vi "Main.vi"() -> ()   [LabVIEW 2026]
doc: "This template is for the Queued Message Handler design pattern.\n\nThe Event Handling Loop generates messages based on user interface actions.\n\nThe Message Handling Loop processes messages generated by the Event Handling Loop, or by other messages. The messages are string values, so new messages can be added easily to the Message Cases case structure in the Message Handling Loop. Each message cluster can also provide an optional value for Message Data, which is a variant that can be converted to whatever message-specific data is required."
uses:
  controls/UI Data.ctl
  support/Message Queue/Enqueue Message (Single).vi
  <vilib>/Utility/error.llb/Error Cluster From Error Code.vi
  <vilib>/ErrorRing/Error Ring.xnode
  support/Message Queue/Message Queue.lvlib
  support/User Event - Stop/User Event - Stop.lvlib
panel:
  out "Slide":dbl(slide) scale=0.0..100.0
  out "Meter":dbl(knob) scale=0.0..10.0
  in  "Volts":dbl(knob) scale=0.0..10.0
  out "Display <Replace Me>":string
  in  "Do Something Else <Replace Me>":bool
  in  "Do Something <Replace Me>":bool
  in  "Exit":bool
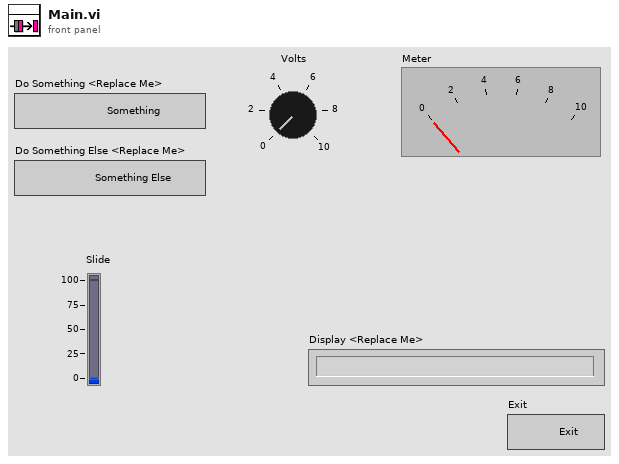
[diagram p1: front panel]
types:
  T1 = typedef "UI Data.ctl" = cluster{"Boolean <Replace Me>":bool, "String <Replace Me>":string, "Numeric <Replace Me>":dbl, "Do Something Ref":refnum<vi>, "Do Something Else Ref":refnum<vi>, "Data Display Ref":refnum<vi>, "Exit Button Ref":refnum<vi>}
  T2 = typedef "Message Queue.lvlib/All Message Queues.ctl" = cluster{"UI":refnum<queue>}
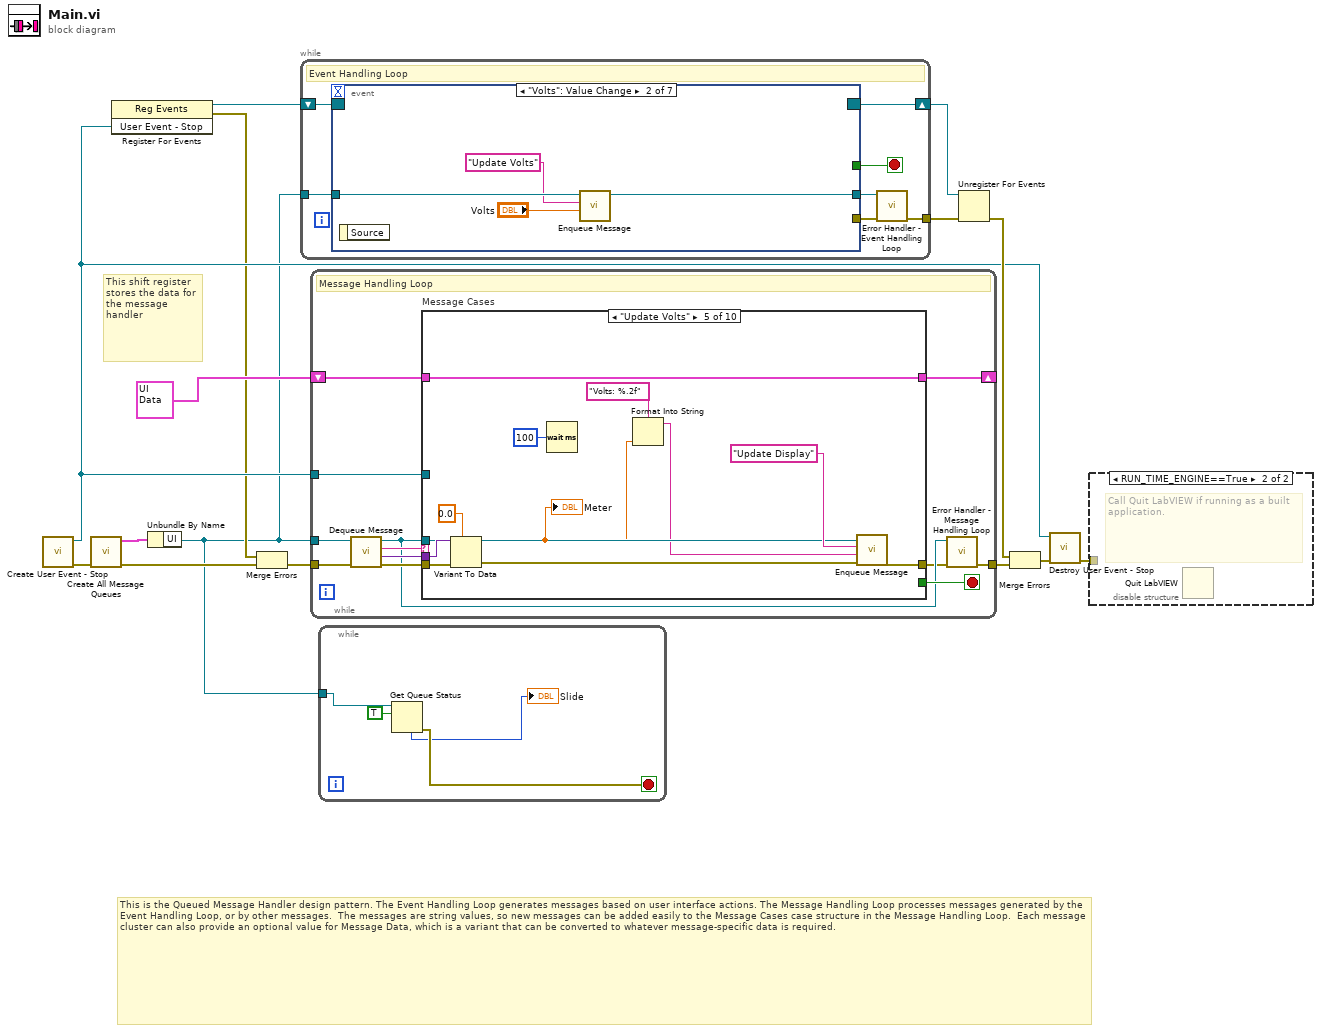
[diagram p0: block diagram]
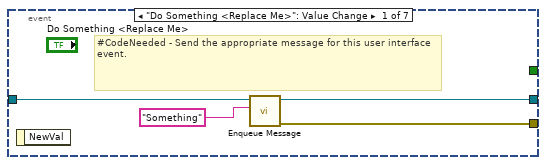
[diagram p3: hidden frame]
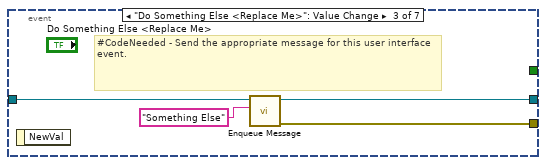
[diagram p4: hidden frame]
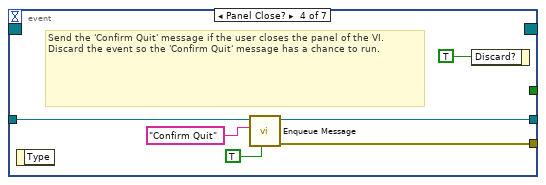
[diagram p5: hidden frame]
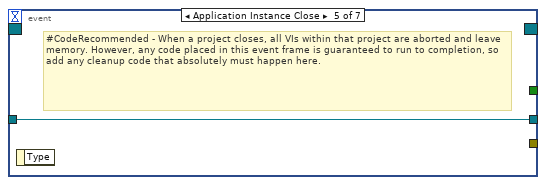
[diagram p6: hidden frame]
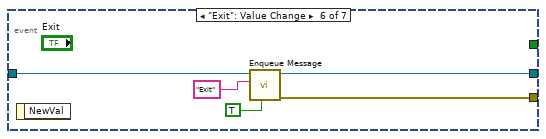
[diagram p7: hidden frame]
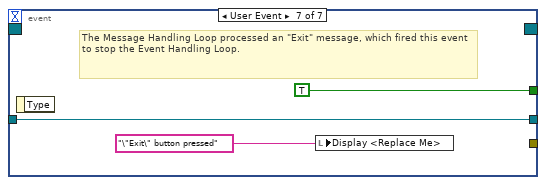
[diagram p8: hidden frame]
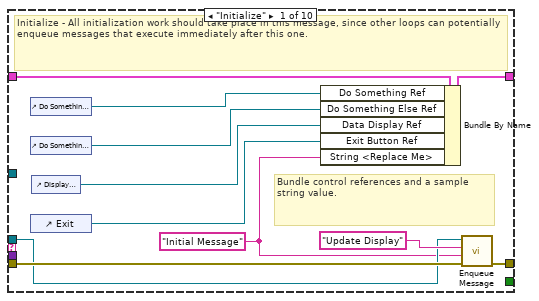
[diagram p9: hidden frame]
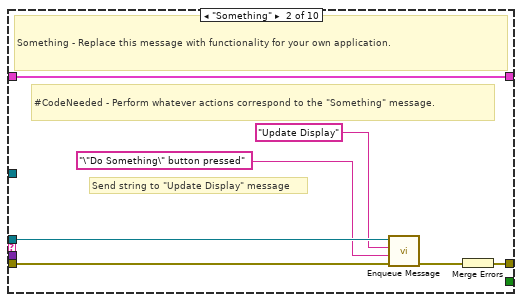
[diagram p10: hidden frame]
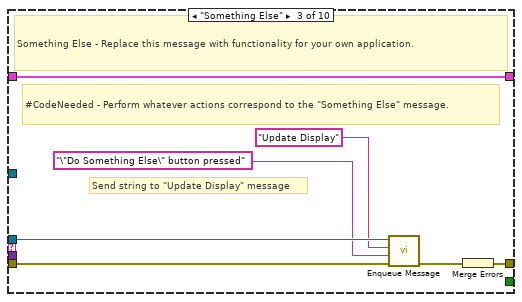
[diagram p11: hidden frame]
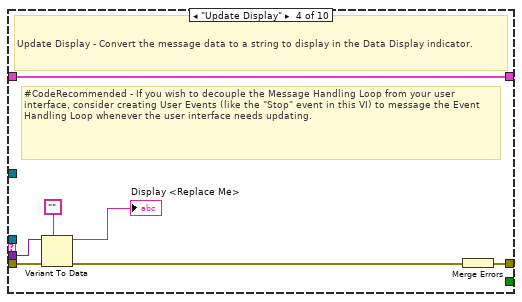
[diagram p12: hidden frame]
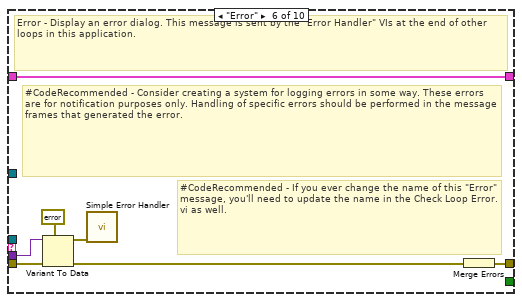
[diagram p13: hidden frame]
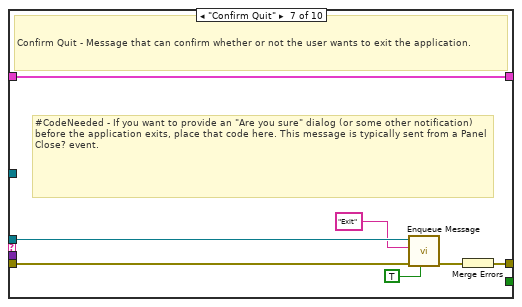
[diagram p14: hidden frame]
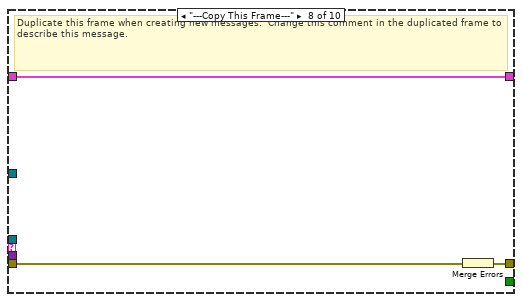
[diagram p15: hidden frame]
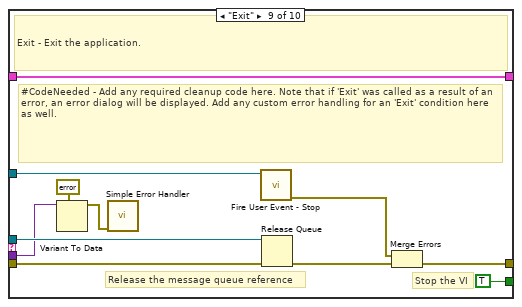
[diagram p16: hidden frame]
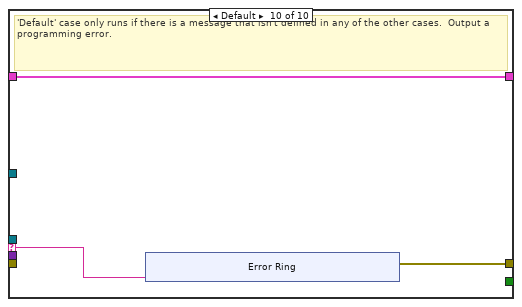
[diagram p17: hidden frame]
diagram:
  # "This is the Queued Message Handler design pattern. The Event Handling Loop generates messages based on user interface actions. The Message Handling Loop processes messages generated by the Event Handling Loop, or by other messages.  The messages are string values, so new messages can be added easily to the Message Cases case structure in the Message Handling Loop.  Each message cluster can also provide an optional value for Message Data, which is a variant that can be converted to whatever message-specific data is required."
  # "This shift register stores the data for the message handler"
  n1 = call "Create User Event - Stop.vi"() -> ("error out"=w12:errorcluster, "User Event - Stop"=w4:refnum<user-event>)  [unwired: 10 in]
  n2 = call "Create All Message Queues.vi"("error in (no error)"=w12) -> ("error out"=w15:errorcluster, "Message Queues out"=w14:T2)  [unwired: 9 in]
  n3 = register-events(w4) -> (reference out=w5:refnum<event-registration>, error out=w2:errorcluster)  [unwired: 2 in]
  n4 = Unbundle By Name(w14) -> ("UI"=w1:refnum<queue>)
  n5 = Merge Errors(w2, w15) -> (w3:errorcluster)
  n6 = while {
    tunnel: w1 -> [w22]
    shift-right: [w20] -> w9
    shift-left: w5 -> [w21]
    tunnel: [w16] -> w6
    stop <- w18 stop-if-true
    # "Event Handling Loop"
    n7 = event shown="[1] \"Volts\": Value Change" {
      selector: w21 -> [_ _ _ _ _ _ _]
      dyn-events: [_ _ _ _ _ _ _] -> w20
      timeout: _ -> [_ _ _ _ _ _ _]
      tunnel: [_ _ _ _ _ _ TRUE ("Discard?")] -> w18
      tunnel: w22 -> [w26 w30 w34 w39 w41 w46 w49]
      tunnel: [w23 _ w31 w38 _ w45 _] -> w19
      tunnel: [w25 w29 w33 w37 w41 w44 w49] -> w17
      event "Do Something <Replace Me>": Value Change {
        # "#CodeNeeded - Send the appropriate message for this user interface event."
        n8 = event-data() -> ()  [unwired: 1 in, 1 out]
        n9 = call-poly "Enqueue Message.vi"("Message"="Something", "Message Queue"=w26) -> ("error out"=w23:errorcluster, "dup Message Queue"=w25:refnum<queue>)  [unwired: 8 in]
      }
      event "Volts": Value Change {
        n10 = event-data() -> ()  [unwired: 1 in, 1 out]
        n11 = call-poly "Enqueue Message.vi"("Message Data"="Volts", "Message"="Update Volts", "Message Queue"=w30) -> ("dup Message Queue"=w29:refnum<queue>)  [unwired: 7 in, 1 out]
      }
      event "Do Something Else <Replace Me>": Value Change {
        # "#CodeNeeded - Send the appropriate message for this user interface event."
        n12 = event-data() -> ()  [unwired: 1 in, 1 out]
        n13 = call-poly "Enqueue Message.vi"("Message"="Something Else", "Message Queue"=w34) -> ("error out"=w31:errorcluster, "dup Message Queue"=w33:refnum<queue>)  [unwired: 8 in]
      }
      event Panel Close? {
        # "Send the 'Confirm Quit' message if the user closes the panel of the VI. Discard the event so the 'Confirm Quit' message has a chance to run."
        n14 = event-data() -> ()  [unwired: 1 in, 1 out]
        n15 = call-poly "Enqueue Message.vi"("Priority Message? (F)"=TRUE, "Message"="Confirm Quit", "Message Queue"=w39) -> ("error out"=w38:errorcluster, "dup Message Queue"=w37:refnum<queue>)  [unwired: 7 in]
        n16 = event-data("Discard?"=TRUE) -> ()  [unwired: 1 in, 1 out]
      }
      event Application Instance Close {
        # "#CodeRecommended - When a project closes, all VIs within that project are aborted and leave memory. However, any code placed in this event frame is guaranteed to run to completion, so add any cleanup code that absolutely must happen here."
        n17 = event-data() -> ()  [unwired: 1 in, 1 out]
      }
      event "Exit": Value Change {
        n18 = event-data() -> ()  [unwired: 1 in, 1 out]
        n19 = call-poly "Enqueue Message.vi"("Priority Message? (F)"=TRUE, "Message"="Exit", "Message Queue"=w46) -> ("error out"=w45:errorcluster, "dup Message Queue"=w44:refnum<queue>)  [unwired: 7 in]
      }
      event User Event {
        # "The Message Handling Loop processed an \"Exit\" message, which fired this event to stop the Event Handling Loop."
        n20 = event-data() -> ()  [unwired: 1 in, 1 out]
        n21 = local write "Display <Replace Me>"("\"Exit\" button pressed" ("VI Stopped")) -> ()
      }
    }
    n22 = call "Error Handler - Event Handling Loop.vi"("error in (no error)"=w19, "Message Queue"=w17) -> ("dup error in"=w16:errorcluster)  [unwired: 8 in, 1 out]
  }
  n23 = while {
    tunnel: w1 -> [w53]
    shift-right: [w60] -> _
    shift-left: T1 {"Boolean <Replace Me>"=FALSE, "String <Replace Me>"="", "Numeric <Replace Me>"=0.0, "Do Something Ref"=refnum, "Do Something Else Ref"=refnum, "Data Display Ref"=refnum, "Exit Button Ref"=refnum} ("Data Cluster") -> [w61]
    tunnel: w4 -> [w58]
    tunnel: w3 -> [w57]
    tunnel: [w51] -> w13
    stop <- w59 stop-if-true
    # "Message Handling Loop"
    n24 = call "Dequeue Message.vi"("error in (no error)"=w57, "Message Queue"=w53) -> ("error out"=w56:errorcluster, "Message Data"=w54:variant, "Message"=w55:string, "dup Message Queue"=w52:refnum<queue>)  [unwired: 6 in]
    n25 = case "Message Cases" shown="\"Update Volts\"" w55 {
      selector: w55 -> [_ _ _ _ _ _ _ _ _ w134]
      tunnel: w52 -> [w63 w75 w82 _ w98 _ w115 _ w133 _]
      tunnel: w56 -> [w71 w77 w84 w91 w105 w112 w119 w122 w126 _]
      tunnel: [w72 w78 w85 w92 w100 w106 w117 w120 w129 w135] -> w50
      tunnel: w61 -> [w70 w79 w86 w93 w104 w111 w118 w121 w132 w136]
      tunnel: [w69 w79 w86 w93 w104 w111 w118 w121 w132 w136] -> w60
      tunnel: [_ _ _ _ _ _ _ _ TRUE _] -> w59
      tunnel: w54 -> [_ _ _ w90 w103 w110 _ _ w123 _]
      tunnel: w58 -> [_ _ _ _ _ _ _ _ w128 _]
      frame "Initialize" {
        w62 = "Initial Message" ("Initial Message")
        # "Bundle control references and a sample string value."
        # "Initialize - All initialization work should take place in this message, since other loops can potentially enqueue messages that execute immediately after this one."
        n26 = control-ref of="Do Something <Replace Me>"() -> (w68:refnum<vi>)
        n27 = control-ref of="Do Something Else <Replace Me>"() -> (w67:refnum<vi>)
        n28 = control-ref of="Exit"() -> (w65:refnum<vi>)
        n29 = control-ref of="Display <Replace Me>"() -> (w66:refnum<vi>)
        n30 = Bundle By Name(cluster=w70, "Do Something Ref"=w68, "Do Something Else Ref"=w67, "Data Display Ref"=w66, "Exit Button Ref"=w65, "String <Replace Me>"=w62) -> (w69:T1)
        n31 = call-poly "Enqueue Message.vi"("error in (no error)"=w71, "Message Data"=w62, "Message"="Update Display", "Message Queue"=w63) -> ("error out"=w72:errorcluster)  [unwired: 6 in, 1 out]
      }
      frame "Something" {
        # "Send string to \"Update Display\" message"
        # "#CodeNeeded - Perform whatever actions correspond to the \"Something\" message."
        # "Something - Replace this message with functionality for your own application."
        n32 = call-poly "Enqueue Message.vi"("error in (no error)"=w77, "Message Data"="\"Do Something\" button pressed" ("\"Do Something\" button pressed"), "Message"="Update Display", "Message Queue"=w75) -> ("error out"=w76:errorcluster)  [unwired: 6 in, 1 out]
        n33 = Merge Errors(w76) -> (w78:errorcluster)
      }
      frame "Something Else" {
        # "Send string to \"Update Display\" message"
        # "#CodeNeeded - Perform whatever actions correspond to the \"Something Else\" message."
        # "Something Else - Replace this message with functionality for your own application."
        n34 = call-poly "Enqueue Message.vi"("error in (no error)"=w84, "Message Data"="\"Do Something Else\" button pressed" ("\"Do Something Else\" button pressed"), "Message"="Update Display", "Message Queue"=w82) -> ("error out"=w83:errorcluster)  [unwired: 6 in, 1 out]
        n35 = Merge Errors(w83) -> (w85:errorcluster)
      }
      frame "Update Display" {
        # "#CodeRecommended - If you wish to decouple the Message Handling Loop from your user interface, consider creating User Events (like the \"Stop\" event in this VI) to message the Event Handling Loop whenever the user interface needs updating."
        # "Update Display - Convert the message data to a string to display in the Data Display indicator."
        n36 = Variant To Data(error in=w91, type="", Variant=w90) -> (data=→"Display <Replace Me>":string, error out=w88:errorcluster)
        n37 = Merge Errors(w88) -> (w92:errorcluster)
      }
      frame "Update Volts" {
        n38 = Variant To Data(error in=w105, type=0.0, Variant=w103) -> (data=w96:dbl, error out=w99:errorcluster)
        "Meter" <- w96
        n39 = Wait (ms)(milliseconds to wait=u32 100) -> ()  [unwired: 1 out]
        n40 = Format Into String(format string="Volts: %.2f", w96) -> (resulting string=w97:string)  [unwired: 2 in, 1 out]
        n41 = call-poly "Enqueue Message.vi"("error in (no error)"=w99, "Message Data"=w97, "Message"="Update Display", "Message Queue"=w98) -> ("error out"=w100:errorcluster)  [unwired: 6 in, 1 out]
      }
      frame "Error" {
        # "#CodeRecommended - If you ever change the name of this \"Error\" message, you'll need to update the name in the Check Loop Error.vi as well."
        # "#CodeRecommended - Consider creating a system for logging errors in some way. These errors are for notification purposes only. Handling of specific errors should be performed in the message frames that generated the error."
        # "Error - Display an error dialog. This message is sent by the \"Error Handler\" VIs at the end of other loops in this application."
        n42 = Variant To Data(error in=w112, type=errorcluster {"status"=FALSE, "code"=0, "source"=""} ("error constant"), Variant=w110) -> (data=w108:errorcluster, error out=w107:errorcluster)
        n43 = call <vilib>:"Simple Error Handler.vi"("error in (no error)"=w108) -> ()  [unwired: 4 in, 5 out]
        n44 = Merge Errors(w107) -> (w106:errorcluster)
      }
      frame "Confirm Quit" {
        # "#CodeNeeded - If you want to provide an \"Are you sure\" dialog (or some other notification) before the application exits, place that code here. This message is typically sent from a Panel Close? event."
        # "Confirm Quit - Message that can confirm whether or not the user wants to exit the application."
        n45 = call-poly "Enqueue Message.vi"("Priority Message? (F)"=TRUE, "error in (no error)"=w119, "Message"="Exit", "Message Queue"=w115) -> ("error out"=w116:errorcluster)  [unwired: 6 in, 1 out]
        n46 = Merge Errors(w116) -> (w117:errorcluster)
      }
      frame "---Copy This Frame---" {
        # "Duplicate this frame when creating new messages.  Change this comment in the duplicated frame to describe this message."
        n47 = Merge Errors(w122) -> (w120:errorcluster)
      }
      frame "Exit" {
        # "Stop the VI"
        # "Release the message queue reference"
        # "#CodeNeeded - Add any required cleanup code here. Note that if 'Exit' was called as a result of an error, an error dialog will be displayed. Add any custom error handling for an 'Exit' condition here as well."
        # "Exit - Exit the application."
        n48 = Variant To Data(type=errorcluster {"status"=FALSE, "code"=0, "source"=""} ("error constant"), Variant=w123) -> (data=w124:errorcluster)  [unwired: 1 in, 1 out]
        n49 = call <vilib>:"Simple Error Handler.vi"("error in (no error)"=w124) -> ()  [unwired: 4 in, 5 out]
        n50 = call "Fire User Event - Stop.vi"("User Event - Stop"=w128) -> ("error out"=w127:errorcluster)  [unwired: 10 in]
        n51 = Release Queue(queue=w133, error in (no error)=w126) -> (error out=w130:errorcluster)  [unwired: 1 in, 2 out]
        n52 = Merge Errors(w127, w130) -> (w129:errorcluster)
      }
      frame Default {
        # "'Default' case only runs if there is a message that isn't defined in any of the other cases.  Output a programming error."
        n53 = xnode "Error Ring"("parameter 0"=w134) -> ("error out"=w135:errorcluster)
      }
    }
    n54 = call "Error Handler - Message Handling Loop.vi"("error in (no error)"=w50, "Message Queue"=w52) -> ("dup error in"=w51:errorcluster)  [unwired: 8 in, 1 out]
  }
  n55 = while {
    tunnel: w1 -> [w147]
    stop <- w146 stop-if-true
    n56 = Get Queue Status(queue=w147, return elements? (F)=TRUE) -> (error out=w146:errorcluster, # elements in queue=→"Slide":i32)  [unwired: 1 in, 6 out]
  }
  n57 = Unregister For Events(event registration refnum=w9, error in=w6) -> (error out=w10:errorcluster)
  n58 = Merge Errors(w10, w13) -> (w11:errorcluster)
  n59 = call "Destroy User Event - Stop.vi"("error in (no error)"=w11, "User Event - Stop"=w4) -> ("error out"=w7:errorcluster)  [unwired: 9 in]
  n60 = disable-structure shown="RUN_TIME_ENGINE==True" {
    disable-tunnel: w7 -> [_ _]
    frame condition #0 (active) {
    }
    frame condition #1 {
      # "Call Quit LabVIEW if running as a built application."
      n61 = Quit LabVIEW() -> ()  [unwired: 1 in]
    }
  }
